vi "video.get_ingest_status.vi"(8 "error in":errorcluster, 10 "Video RID":string, 11 "Nominal Client in":refnum<class "Nominal Client.lvclass">) -> (0 "error out":errorcluster, 1 "Progress (0-1)":dbl, 2 "Status":string, 3 "Nominal Client out":refnum<class "Nominal Client.lvclass">)   [LabVIEW 2020, in "Nominal Client.lvclass"]
doc: "The returned status will be:\nsuccess, error, or inProgress"
uses:
  Nominal Client.lvclass
  Nominal Client.lvclass/Nominal Client.ctl
  3ce23808-1dd2-45d8-8215-d591b3b9a39c.vi
  create.authorization_header.vi
  trace.payload_sent.vi
  trace.payload_received.vi
  error.vi
  api_token.get.vi
  trace.generate.vi
  <vilib>/AdvancedString/1D String Array to Delimited String.vi
  <vilib>/JDP Science/JDP Science Common Utilities/Trim Whitespace__JDP.vi
  trace.calling_method.vi
  error.vi/859f8e04-e495-489b-b5b4-7ac163f56130.vi
  <vilib>/Utility/libraryn.llb/Get File Extension.vi
  log_file.write.vi
  <vilib>/JDP Science/JSONtext/Get all Object Items.vi
  <vilib>/JDP Science/JSONtext/JSON text to Variant.vi
  <vilib>/JDP Science/JSONtext/LVClass Serializer/JSONtext LVClass Serializer.lvclass
  <vilib>/addons/_JKI.lib/REST Client/classes/Response Headers/Response Headers.lvclass
  <vilib>/addons/_JKI.lib/REST Client/classes/REST Client/REST Client.lvclass
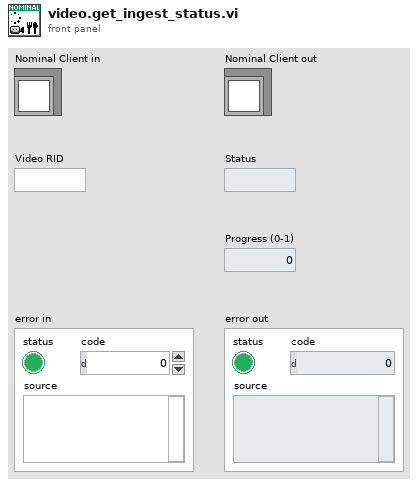
[diagram p1: front panel]
types:
  T1 = cluster{"type":string, "error":cluster{"errors":cluster{"errorType":string, "message":string}[]}, "inProgress":dbl}
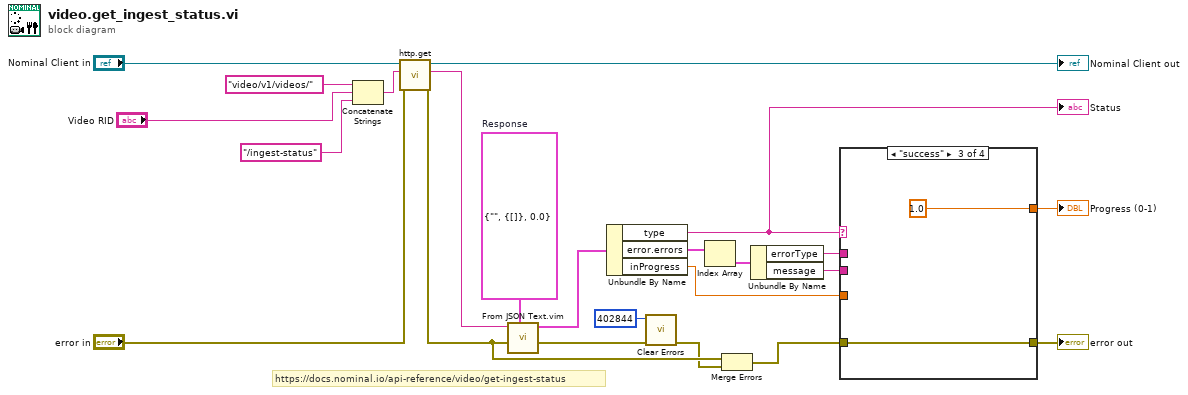
[diagram p0: block diagram]
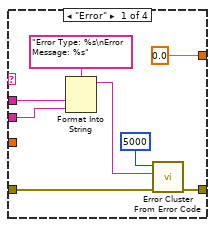
[diagram p2: hidden frame]
diagram:
  w11 = T1 {"type"="", "error"={"errors"=[]}, "inProgress"=0.0}  # Response
  # "https://docs.nominal.io/api-reference/video/get-ingest-status"
  n1 = Concatenate Strings("video/v1/videos/" ("Path"), "Video RID", "/ingest-status" ("Path")) -> (w21:string)
  n2 = call "http.get.vi"("error in"="error in", "Path"=w21, "Nominal Client in"="Nominal Client in") -> ("error out"=w3:errorcluster, "Response"=w18:string, "Nominal Client out"=→"Nominal Client out":refnum<class "Nominal Client.lvclass">)  [unwired: 5 in, 1 out]
  n3 = call "From JSON Text.vim"("Data Type and Default Value"=w11, "error in (no error)"=w3, "JSON"=w18) -> ("error out"=w19:errorcluster, "Data out"=w17:T1)  [unwired: 7 in]
  n4 = Unbundle By Name(w17) -> ("type"=w6:string, "error.errors"=w10:cluster{"errorType":string, "message":string}[], "inProgress"=w4:dbl)
  "Status" <- w6
  n5 = call <vilib>:"Clear Errors.vi"("error in (no error)"=w19, "specific error code to clear (0: all)"=402844) -> ("error out"=w2:errorcluster)  [unwired: 4 in, 1 out]
  n6 = Index Array(array=w10) -> (element=w9:cluster{"errorType":string, "message":string})  [unwired: 1 in]
  n7 = Merge Errors(w3, w2) -> (w1:errorcluster)
  n8 = Unbundle By Name(w9) -> ("errorType"=w8:string, "message"=w7:string)
  n9 = case shown="\"success\"" w6 {
    tunnel: w1 -> [w30 w32 w34 w36]
    tunnel: [w31 w32 w34 w36] -> w12
    tunnel: w8 -> [w26 _ _ _]
    tunnel: w7 -> [w25 _ _ _]
    tunnel: [0.0 w33 1.0 _] -> w5
    tunnel: w4 -> [_ w33 _ _]
    frame "Error" {
      n10 = Format Into String(format string="Error Type: %s\nError Message: %s", w26, w25) -> (resulting string=w27:string)  [unwired: 2 in, 1 out]
      n11 = call <vilib>:"Error Cluster From Error Code.vi"("error in (no error)"=w30, "error message (\"\")"=w27, "error code (0)"=5000) -> ("error out"=w31:errorcluster)  [unwired: 6 in]
    }
    frame "inProgress" {
    }
    frame "success" {
    }
    frame Default {
    }
  }
  "error out" <- w12
  "Progress (0-1)" <- w5
